vi "ReplaceSelf.vi"(0 "XRef":T9, 1 "Terms":T6, 2 "Diagram":T5, 3 "State In":T4) -> (14 "Replace Self?":T1, 15 "Reply":T2)   [LabVIEW 2012, in "OpenG FilterArray.xnode"]
doc: "This ability VI is called when you want to replace this XNode via LabVIEW's scripting API. This VI is only called when you have previously informed LabVIEW that you want to replace the XNode through a ReplaceSelf reply. Diagram is a reference to a diagram of a temporary VI. This diagram contains exactly one front panel terminal for each terminal of your XNode. Terms is an array of pairs of Term IDs and terminal references. LabVIEW will replace your XNode with code scripted into this diagram into the diagram of the VI containing your XNode and connect everything to the correct terminals. The front panel terminals that are on this diagram are special in that they can only be on the top level diagram.\n \n Replace Self? is used to tell LabVIEW whether or not you want to copy the scripted diagram over. If there is an error and you wish not to commit the changes, then the old XNode behavior will be left unchanged. It will not be called again until you indicate that it should be through the reply on another ability VI.\n \n You should not use the Copy scripting method to move code into the temporary VI. This will adversely affect the user's clipboard. You should use the Move scripting method instead.\n\nDefault behavior: None.\n\nThis ability does not provide UI and OS messages are not handled.\n\nSee also: AugmentSelf"
uses:
  OpenG FilterArray.xnode
  <vilib>/XNodeSupport/XNodeXNodeRef.ctl
  <vilib>/XNodeSupport/XNodeTermIDPairs.ctl
  <vilib>/XNodeSupport/XNodeTermIDPair.ctl
  <vilib>/XNodeSupport/XNodeTermRef.ctl
  <vilib>/XNodeSupport/XNodeString.ctl
  <vilib>/XNodeSupport/XNodeTopLevelDiagramRef.ctl
  State.ctl
  <vilib>/XNodeSupport/XNodeStringArray.ctl
  <vilib>/XNodeSupport/XNodeBool.ctl
  <vilib>/Utility/miscctls.llb/LVPositionTypeDef.ctl
  <userlib>/_LAVAcr/Scripting Tools/Scripting Tools.lvlib
  <vilib>/XNodeSupport/NI_XNodeSupport.lvlib
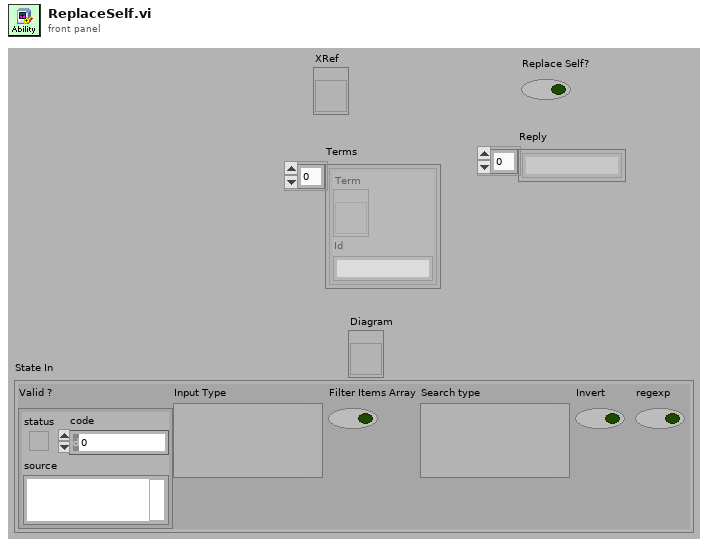
[diagram p1: front panel]
types:
  T1 = typedef "NI_XNodeSupport.lvlib/XNodeBool.ctl" = bool
  T2 = typedef "NI_XNodeSupport.lvlib/XNodeStringArray.ctl" = T3[]
  T3 = typedef "NI_XNodeSupport.lvlib/XNodeString.ctl" = string
  T4 = typedef "OpenG FilterArray.xnode/State.ctl" = cluster{"Valid ?":errorcluster, "Input Type":variant, "Filter Items Array":bool, "Search type":variant, "Invert":bool, "regexp":bool}
  T5 = typedef "NI_XNodeSupport.lvlib/XNodeTopLevelDiagramRef.ctl" = refnum<vi>
  T6 = typedef "NI_XNodeSupport.lvlib/XNodeTermIDPairs.ctl" = T7[]
  T7 = typedef "NI_XNodeSupport.lvlib/XNodeTermIDPair.ctl" = cluster{"Term":T8, "Id":T3}
  T8 = typedef "NI_XNodeSupport.lvlib/XNodeTermRef.ctl" = refnum<vi>
  T9 = typedef "NI_XNodeSupport.lvlib/XNodeXNodeRef.ctl" = refnum<vi>
  T10 = typedef "LVPositionTypeDef.ctl" = cluster{"Left":i32, "Top":i32}
  T11 = cluster{"Alignment":enum32{"Left", "Right", "Hybrid", "Center", "Gravity"}, "Rules":enum32{"Strict", "Allow Wires Under Labels", "Allow Wires Under Lead Nodes", "Allow Wires Under Wide Blocks"}, "Max Heuristic Iterations":u32, "Max Simplex Iterations":u32, "Block Padding":cluster{"Horizontal":i32, "Vertical":i32}, "Wire Padding":cluster{"Horizontal":i32, "Vertical":i32}, "Auto-Tune by Topology":bool, "Fine-Tune Y Positions":bool, "Align All Controls on Left":bool, "Align All Indicators on Right":bool, "Use Array Dimension Heuristics":bool}
  T12 = typedef "imagedata.ctl" = cluster{"image type":i32, "image depth":i32, "image":u8[], "mask":u8[], "colors":u32[], "Rectangle":cluster{"left":i16, "top":i16, "right":i16, "bottom":i16}}
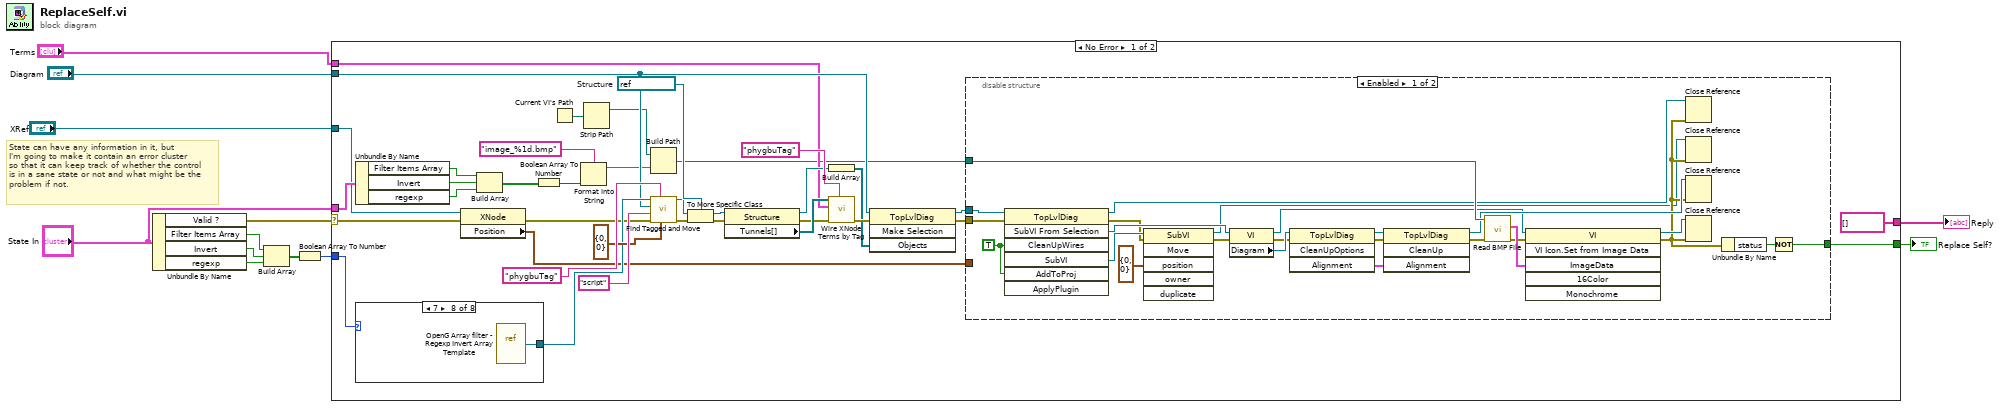
[diagram p0: block diagram]
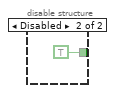
[diagram p2: hidden frame]
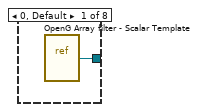
[diagram p3: hidden frame]
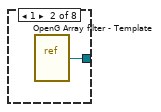
[diagram p4: hidden frame]
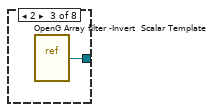
[diagram p5: hidden frame]
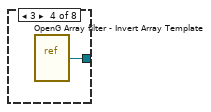
[diagram p6: hidden frame]
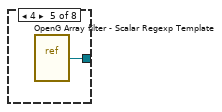
[diagram p7: hidden frame]
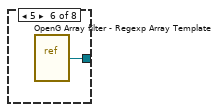
[diagram p8: hidden frame]
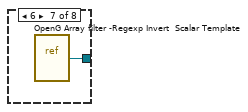
[diagram p9: hidden frame]
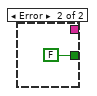
[diagram p10: hidden frame]
diagram:
  # "State can have any information in it, but\nI'm going to make it contain an error cluster\nso that it can keep track of whether the control\nis in a sane state or not and what might be the\nproblem if not."
  n1 = Unbundle By Name("State In") -> ("Valid ?"=w12:errorcluster, "Filter Items Array"=w10:bool, "Invert"=w9:bool, "regexp"=w7:bool)
  n2 = Build Array(w10, w9, w7) -> (w11:bool[])
  n3 = Boolean Array To Number(Boolean array=w11) -> (number=w8:u32)
  n4 = case shown="No Error" w12 {
    selector: w12 -> [w15 _]
    tunnel: "State In" -> [w17 _]
    tunnel: "Diagram" -> [w34 _]
    tunnel: "Terms" -> [w28 _]
    tunnel: [string[] [] ("Reply") _] -> w2
    tunnel: [w35 FALSE] -> w3
    tunnel: w8 -> [w37 _]
    tunnel: "XRef" -> [w16 _]
    frame No Error {
      w47 = refnum<vi> refnum  # Structure
      n5 = Unbundle By Name(w17) -> ("Filter Items Array"=w24:bool, "Invert"=w23:bool, "regexp"=w22:bool)
      n6 = case shown="7" w37 {
        tunnel: [w76 w77 w78 w79 w80 w81 w82 w83] -> w36
        frame 0, Default {
          n7 = vi-ref "OpenG Array filter - Scalar Template.vi"() -> (w76:refnum<vi>)
        }
        frame 1 {
          n8 = vi-ref "OpenG Array filter - Template.vi"() -> (w77:refnum<vi>)
        }
        frame 2 {
          n9 = vi-ref "OpenG Array filter -Invert  Scalar Template.vi"() -> (w78:refnum<vi>)
        }
        frame 3 {
          n10 = vi-ref "OpenG Array filter - Invert Array Template.vi"() -> (w79:refnum<vi>)
        }
        frame 4 {
          n11 = vi-ref "OpenG Array filter - Scalar Regexp Template.vi"() -> (w80:refnum<vi>)
        }
        frame 5 {
          n12 = vi-ref "OpenG Array filter - Regexp Array Template.vi"() -> (w81:refnum<vi>)
        }
        frame 6 {
          n13 = vi-ref "OpenG Array filter -Regexp Invert  Scalar Template.vi"() -> (w82:refnum<vi>)
        }
        frame 7 {
          n14 = vi-ref "OpenG Array filter - Regexp Invert Array Template.vi"() -> (w83:refnum<vi>)
        }
      }
      n15 = property class="XNode"(reference=w16, error in=w15) -> (error out=w14:errorcluster, "Position"=w13:T10)  [unwired: 1 out]
      n16 = Build Array(w24, w23, w22) -> (w21:bool[])
      n17 = Boolean Array To Number(Boolean array=w21) -> (number=w19:u32)
      n18 = Current VI's Path() -> (path=w27:path)
      n19 = Format Into String(format string="image_%1d.bmp" ("name or relative path"), w19) -> (resulting string=w18:string)  [unwired: 2 in, 1 out]
      n20 = Strip Path(path=w27) -> (stripped path=w26:path)  [unwired: 1 out]
      n21 = Build Path(base path=w26, name or relative path=w18) -> (appended path=w25:path)
      n22 = call <userlib>:"Find Tagged and Move.vi"("position"=T10 {"Left"=0, "Top"=0}, "TagName"="phygbuTag", "error in"=w14, "TagValue"="script", "Destination Diagram"=w34, "VI Refnum"=w36) -> ("error out"=w41:errorcluster, "Moved Tagged object"=w42:refnum<vi>)  [unwired: 4 out]
      n23 = To More Specific Class(target class=w47, reference=w42, error in=w41) -> (specific class reference=w48:refnum<vi>, error out=w40:errorcluster)
      n24 = property class="Structure"(reference=w48, error in=w40) -> (reference out=w32:refnum<vi>, error out=w39:errorcluster, "Tunnels[]"=w46:refnum<vi>[])
      n25 = Build Array(w32) -> (w31:refnum<vi>[])
      n26 = call <userlib>:"Wire XNode Terms by Tag.vi"("TagName"="phygbuTag", "error in (no error)"=w39, "Term Refs"=w28, "Source References"=w46) -> ("error out"=w33:errorcluster)  [unwired: 7 out]
      n27 = invoke class="TopLvlDiag" method="Make Selection"(reference=w34, error in=w33, "Objects"=w31) -> (reference out=w29:T5, error out=w30:errorcluster)  [unwired: 1 in, 2 out]
      n28 = disable-structure shown="Enabled" {
        disable-tunnel: [w72 TRUE] -> w35
        disable-tunnel: w30 -> [w71 _]
        disable-tunnel: w29 -> [w70 _]
        disable-tunnel: w25 -> [w69 _]
        disable-tunnel: w13 -> [_ _]
        frame Enabled {
          w74 = TRUE ("Clean Up Wires")
          n29 = invoke class="TopLvlDiag" method="SubVI From Selection"(reference=w70, error in=w71, "CleanUpWires"=w74, "AddToProj"=w74) -> (reference out=w57:T5, error out=w54:errorcluster, "SubVIFromSelection"=w66:refnum<vi>, "SubVI"=w55:refnum<vi>)  [unwired: 3 in, 3 out]
          n30 = invoke class="SubVI" method="Move"(reference=w55, error in=w54, "position"=T10 {"Left"=0, "Top"=0}) -> (reference out=w52:refnum<vi>, error out=w53:errorcluster)  [unwired: 3 in, 4 out]
          n31 = property class="VI"(reference=w66, error in=w53) -> (reference out=w51:refnum<vi>, error out=w61:errorcluster, "Diagram"=w64:refnum<vi>)
          n32 = invoke class="TopLvlDiag" method="CleanUpOptions"(reference=w64, error in=w61) -> (reference out=w63:refnum<vi>, error out=w60:errorcluster, "Alignment"=w62:T11)  [unwired: 2 in, 1 out]
          n33 = invoke class="TopLvlDiag" method="CleanUp"(reference=w63, error in=w60, "Alignment"=w62) -> (reference out=w58:refnum<vi>, error out=w65:errorcluster)  [unwired: 1 in, 2 out]
          n34 = call <vilib>:"Read BMP File.vi"("error in (no error)"=w65, "path to BMP file"=w69) -> ("error out"=w67:errorcluster, "image data"=w68:T12)  [unwired: 8 out]
          n35 = invoke class="VI" method="VI Icon.Set from Image Data"(reference=w51, error in=w67, "ImageData"=w68) -> (reference out=w59:refnum<vi>, error out=w56:errorcluster)  [unwired: 3 in, 4 out]
          n36 = Close Reference(reference=w57, error in (no error)=w56) -> ()  [unwired: 1 out]
          n37 = Close Reference(reference=w52, error in (no error)=w56) -> ()  [unwired: 1 out]
          n38 = Close Reference(reference=w58, error in (no error)=w56) -> ()  [unwired: 1 out]
          n39 = Close Reference(reference=w59, error in (no error)=w56) -> ()  [unwired: 1 out]
          n40 = Unbundle By Name(w56) -> ("status"=w73:bool)
          n41 = Not(x=w73) -> (.not. x?=w72:bool)
        }
        frame Disabled {
        }
      }
    }
    frame Error {
    }
  }
  "Reply" <- w2
  "Replace Self?" <- w3
